vi "Read.vi"(8 "error in (no error)":errorcluster, 11 "Concatenate_STR in":refnum<class "Concatenate_STR.lvclass">) -> (0 "error out":errorcluster, 2 "String":string, 3 "Concatenate_STR out":refnum<class "Concatenate_STR.lvclass">)   [LabVIEW 2021, in "Concatenate_STR.lvclass"]
uses:
  Concatenate_STR.lvclass
  Concatenate_STR.lvclass/Concatenate_STR.ctl
  Abs_Types/Value/Abs_Value.lvclass
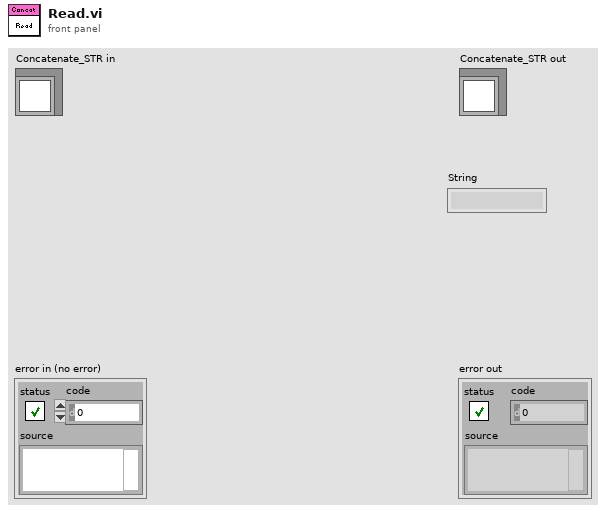
[diagram p1: front panel]
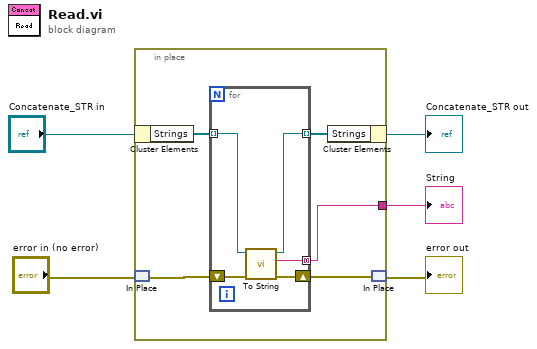
[diagram p0: block diagram]
diagram:
  n1 = in-place {
    in-place-border: [w6] -> w1
    n2 = in-place-cluster #1("Concatenate_STR in") -> ("Strings"=w9:refnum<class "Abs_Value.lvclass">[])
    n3 = in-place-match #2("error in (no error)") -> (w10:errorcluster)
    n4 = for {
      tunnel: w9 -> [w14] mode=indexing
      tunnel: [w13] -> w8 mode=indexing
      shift-right: [w12] -> w7
      shift-left: w10 -> [w15]
      tunnel: [w11] -> w6 mode=concatenating
      n5 = call-dynamic "To String.vi"("error in (no error)"=w15, "Types in"=w14) -> ("error out"=w12:errorcluster, "String"=w11:string, "Types out"=w13:refnum<class "Abs_Value.lvclass">)  [unwired: 7 in]
    }
    n6 = in-place-cluster #1("Strings"=w8) -> (→"Concatenate_STR out":refnum<class "Concatenate_STR.lvclass">)
    n7 = in-place-match #2(w7) -> (→"error out":errorcluster)
  }
  "String" <- w1
